vi "Difference Quotient (multiple).vi"(6 "Interval Units (points)":enum16{"Points", "Data"}(ring), 8 "error in (no error)":errorcluster, 9 "Type":enum16{"y/x vs x", "x/y vs y"}(ring), 10 "Window [h] (2)":dbl=2.0 min=2.0, 11 "XY-data":cluster{"X-array":dbl[], "Y-array":dbl[]}[](array[cluster]) {"Y-array" format="%.2p"; "X-array" format="%.2p"}) -> (0 "error out":errorcluster, 2 "Difference Quotient":cluster{"X-array":dbl[], "Y-array":dbl[]}[](array[cluster]), 3 "XY-data out":cluster{"X-array":dbl[], "Y-array":dbl[]}[](array[cluster]) {"Y-array" format="%.2p"; "X-array" format="%.2p"})   [LabVIEW 2019, in "xy_utilities.lvlib"]
doc: "Calculate the difference quotient (y[i-h/2]-y[i+h/s])/(x[i-h/2]-x[i+h/2]).\n\nWire data to the data input to determine the polymorphic instance to use or manually select the instance."
uses:
  xy_utilities.lvlib
  Swap X and Y.vi
  Swap X and Y (single).vi
  Private/X Units.vi
  Private/DQ subVI.vi
  Reverse.vi
  Reverse (single).vi
  Divide.vi
  Divide float (single).vi
  Add.vi
  Add XY (single).vi
  Private/X Array Range to Index.vi
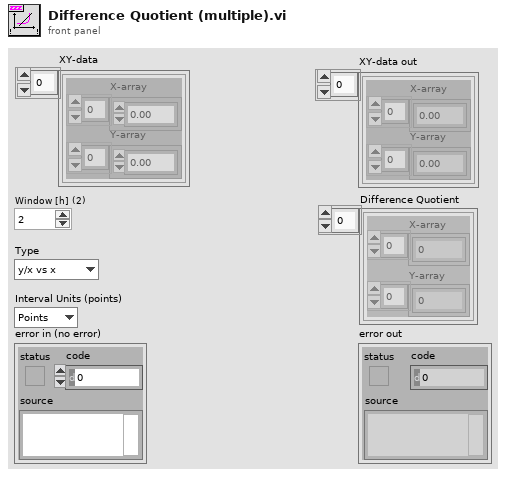
[diagram p1: front panel]
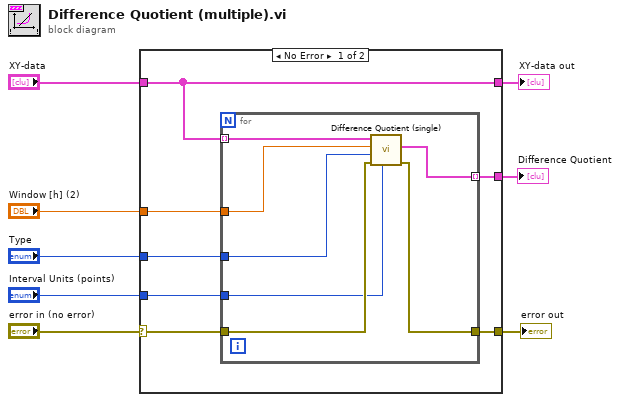
[diagram p0: block diagram]
diagram:
  n1 = case shown="No Error" "error in (no error)" {
    selector: "error in (no error)" -> [w15 w24]
    tunnel: [w14 w24] -> w7
    tunnel: "XY-data" -> [w9 w23]
    tunnel: [w9 w23] -> w5
    tunnel: "Type" -> [w13 _]
    tunnel: "Window [h] (2)" -> [w12 _]
    tunnel: [w11 _] -> w2
    tunnel: "Interval Units (points)" -> [w10 _]
    frame No Error {
      n2 = for {
        tunnel: w9 -> [w22] mode=indexing
        tunnel: w13 -> [w16]
        tunnel: w12 -> [w18]
        tunnel: [w21] -> w11 mode=indexing
        tunnel: w10 -> [w17]
        tunnel: w15 -> [w20]
        tunnel: [w19] -> w14
        n3 = call "Difference Quotient (single).vi"("Interval Units (points)"=w17, "error in (no error)"=w20, "Type"=w16, "Window [h] (2)"=w18, "XY-data"=w22) -> ("error out"=w19:errorcluster, "Difference Quotient"=w21:cluster{"X-array":dbl[], "Y-array":dbl[]})  [unwired: 4 in, 1 out]
      }
    }
    frame Error {
    }
  }
  "error out" <- w7
  "XY-data out" <- w5
  "Difference Quotient" <- w2
